vi "Build table.vi"(7 "Limit (10k)":i32=10000 format="%.0p", 8 "error in":errorcluster, 9 "Tree Data":refnum<vi>, 10 "New Data in":string[][](array[string]), 11 "Tree Data in":string[][](array[string])) -> (0 "error out":errorcluster, 3 "Tree Data out":string[][](array[string]))   [LabVIEW 2025, in "CAN-LIN Raw Bus Capture UI.lvlib"]
uses:
  CAN-LIN Raw Bus Capture UI.lvlib
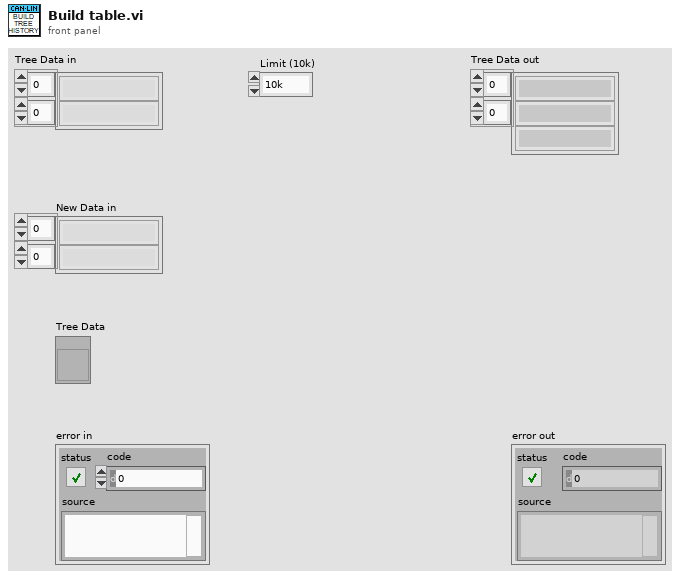
[diagram p1: front panel]
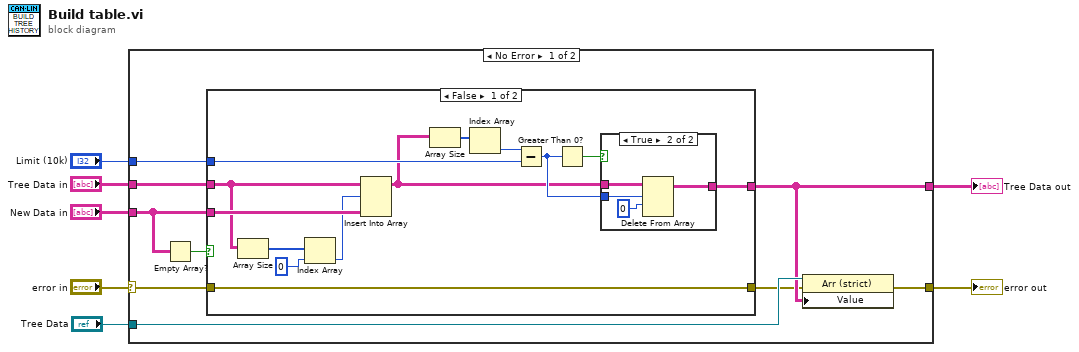
[diagram p0: block diagram]
diagram:
  n1 = case shown="No Error" "error in" {
    selector: "error in" -> [w12 w38]
    tunnel: "New Data in" -> [w15 _]
    tunnel: [w9 w38] -> w5
    tunnel: "Limit (10k)" -> [w14 _]
    tunnel: "Tree Data in" -> [w13 w37]
    tunnel: [w10 w37] -> w2
    tunnel: "Tree Data" -> [w11 _]
    frame No Error {
      n2 = Empty Array?(array=w15) -> (empty?=w16:bool)
      n3 = case shown="False" w16 {
        tunnel: w15 -> [w26 _]
        tunnel: [w23 w36] -> w8
        tunnel: w14 -> [w29 _]
        tunnel: w13 -> [w20 w35]
        tunnel: [w22 w35] -> w10
        tunnel: w12 -> [w23 w36]
        frame False {
          n4 = Array Size(array=w20) -> (size(s)=w19:i32[])
          n5 = Index Array(array=w19, index=0) -> (element=w17:i32)
          n6 = Insert Into Array(array=w20, index (row)=w17, new element=w26) -> (w21:string[][])  [unwired: 1 in]
          n7 = Array Size(array=w21) -> (size(s)=w25:i32[])
          n8 = Index Array(array=w25) -> (element=w24:i32)  [unwired: 1 in]
          n9 = Subtract(x=w24, y=w29) -> (x-y=w27:i32)
          n10 = Greater Than 0?(x=w27) -> (x > 0?=w28:bool)
          n11 = case shown="True" w28 {
            tunnel: [w30 w34] -> w22
            tunnel: w27 -> [_ w33]
            tunnel: w21 -> [w30 w31]
            frame False {
            }
            frame True {
              n12 = Delete From Array(array=w31, length=w33, index (row)=0) -> (array with subset deleted=w34:string[][])  [unwired: 1 in, 1 out]
            }
          }
        }
        frame True {
        }
      }
      n13 = property class="Arr (strict)"(reference=w11, error in=w8, "Value"=w10) -> (error out=w9:errorcluster)  [unwired: 1 out]
    }
    frame Error {
    }
  }
  "error out" <- w5
  "Tree Data out" <- w2
